vi "Test HTTP Header Read Timeout.vi"(8 "error in (no error)":errorcluster, 11 "TestCase in":refnum<class "Test WebSockets Core.lvclass">) -> (0 "error out":errorcluster, 3 "TestCase out":refnum<class "Test WebSockets Core.lvclass">)   [LabVIEW 2013, in "Test WebSockets Core.lvclass"]
uses:
  Test WebSockets Core.lvclass
  WebSockets/WebSocket Server/WebSocket Server.lvclass
  <vilib>/addons/_JKI Toolkits/VI Tester/TestCase.llb/TestCase.lvclass
  WebSockets/WebSocket/WebSocket.lvclass
  Sockets/VISA TCP Socket/VISA TCP.lvclass
panel:
  out "Read time":u32
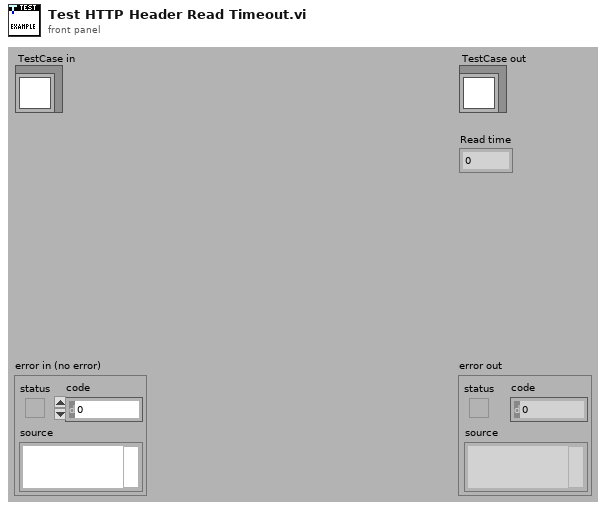
[diagram p1: front panel]
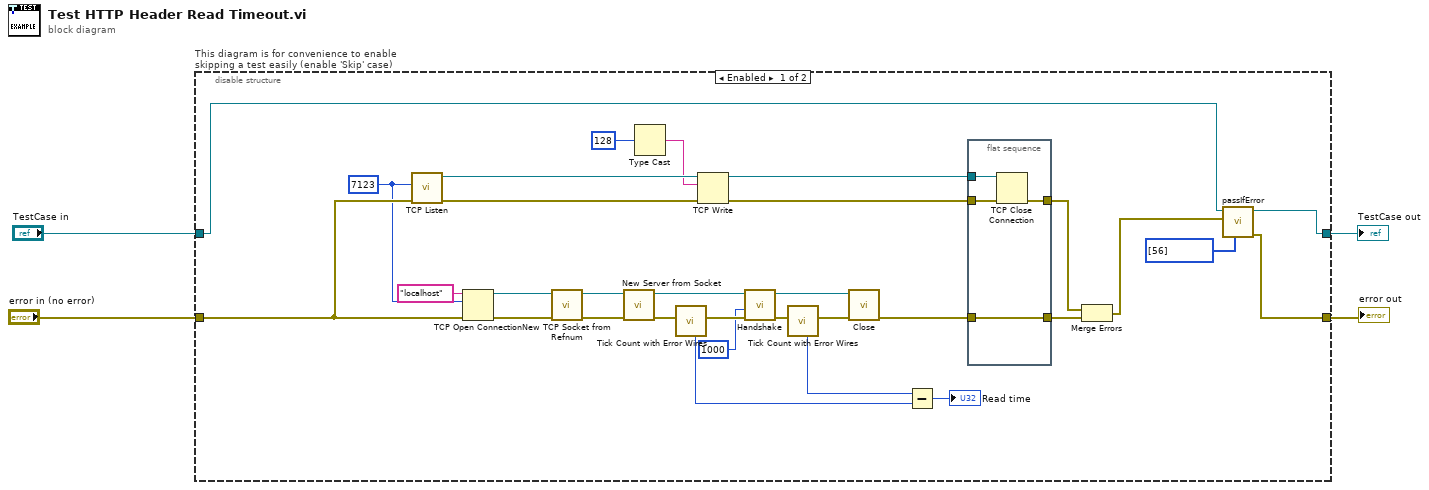
[diagram p0: block diagram]
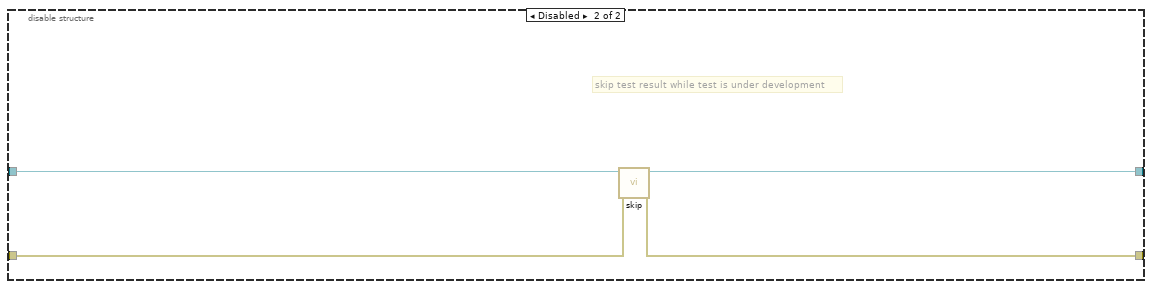
[diagram p2: hidden frame]
diagram:
  n1 = disable-structure "This diagram is for convenience to enable skipping a test easily (enable 'Skip' case)" shown="Enabled" {
    disable-tunnel: "TestCase in" -> [w7 w43]
    disable-tunnel: [w8 w41] -> w1
    disable-tunnel: [w5 w42] -> w3
    disable-tunnel: "error in (no error)" -> [w35 w40]
    frame Enabled {
      w34 = u16 7123 ("port")
      n2 = call <vilib>:"TCP Listen.vi"("error in (no error)"=w35, "port"=w34) -> ("error out"=w32:errorcluster, "connection ID"=w31:refnum<k5>)  [unwired: 5 in, 3 out]
      n3 = TCP Open Connection(address="localhost", remote port or service name=w34, error in (no error)=w35) -> (connection ID=w12:refnum<k5>, error out=w13:errorcluster)  [unwired: 2 in]
      n4 = call "New TCP Socket from Refnum.vi"("error in (no error)"=w13, "TCP Network Connection Refnum"=w12) -> ("error out"=w10:errorcluster, "VISA TCP out"=w11:refnum<class "VISA TCP.lvclass">)  [unwired: 8 in]
      n5 = call "New Server from Socket.vi"("error in (no error)"=w10, "Socket"=w11) -> ("error out"=w14:errorcluster, "WebSocket Server out"=w15:refnum<class "WebSocket Server.lvclass">)  [unwired: 8 in]
      n6 = Type Cast(x=u8 128) -> (*(type *) &x=w29:string)  [unwired: 1 in]
      n7 = call "Tick Count with Error Wires.vi"("error in (no error)"=w14) -> ("error out"=w20:errorcluster, "millisecond timer value"=w22:u32)  [unwired: 9 in]
      n8 = TCP Write(connection ID=w31, data in=w29, error in (no error)=w32) -> (connection ID out=w25:refnum<k5>, error out=w26:errorcluster)  [unwired: 1 in, 1 out]
      n9 = call-dynamic "Handshake.vi"("error in (no error)"=w20, "timeout ms (5000)"=1000, "WebSocket Connection in"=w15) -> ("error out"=w19:errorcluster, "WebSocket Connection out"=w16:refnum<class "WebSocket Server.lvclass">)  [unwired: 7 in]
      n10 = call "Tick Count with Error Wires.vi"("error in (no error)"=w19) -> ("error out"=w24:errorcluster, "millisecond timer value"=w23:u32)  [unwired: 9 in]
      n11 = call-dynamic "Close.vi"("error in (no error)"=w24, "WebSocket in"=w16) -> ("error out"=w17:errorcluster)  [unwired: 9 in]
      n12 = Subtract(x=w23, y=w22) -> (x-y=→"Read time":u32)
      n13 = flat-sequence {
        tunnel: w17 -> [w39]
        tunnel: [w39] -> w28
        tunnel: [w38] -> w27
        tunnel: w26 -> [w37]
        tunnel: w25 -> [w36]
        frame #0 {
          n14 = TCP Close Connection(connection ID=w36, error in (no error)=w37) -> (error out=w38:errorcluster)  [unwired: 1 in, 1 out]
        }
      }
      n15 = Merge Errors(w27, w28) -> (w6:errorcluster)
      n16 = call-dynamic "passIfError.vi"("passing error codes (default = any error code)"=i32[] [56], "error"=w6, "TestCase in"=w7) -> ("error out"=w5:errorcluster, "TestCase out"=w8:refnum<class "Test WebSockets Core.lvclass">)  [unwired: 7 in]
    }
    frame Disabled {
      # "skip test result while test is under development"
      n17 = call <vilib>:"skip.vi"("error in (no error)"=w40, "TestCase in"=w43) -> ("error out"=w42:errorcluster, "TestCase out"=w41:refnum<class "Test WebSockets Core.lvclass">)  [unwired: 8 in]
    }
  }
  "error out" <- w3
  "TestCase out" <- w1
